vi "Test Explorer.vi"() -> ()   [LabVIEW 2017, in "Test Explorer.lvlib"]
uses:
  Test Explorer.lvlib
  Test Case/Test Case.lvclass
  Test Result/Test Result.lvclass
  Test Executor/Test Executor.lvclass
  Code Coverage/Code Coverage.lvclass
  LVUnit Test Discoverer/LVUnit Test Discoverer.lvclass
  LVUnit Test Executor/LVUnit Test Executor.lvclass
  C:/Users/pasca/Projects/Home/lvunit/Test Executor/Test Executor.lvclass
  Test Case/Test Case.lvclass/Test Case.ctl
  Test Outcome.ctl
  Test Executor/Test Executor.lvclass/Test Executor.ctl
  Test Result/Test Result.lvclass/Test Result.ctl
  <vilib>/Utility/sysdir.llb/System Directory Type.ctl
  Test Case/Get Qualified Name.vi
  Test Result/Get Outcome.vi
  Test Executor/Read Result Queue.vi
  Test Executor/Read Application.vi
  Cobertura/Project Inspector/Project Inspector.lvclass
  C:/Users/pasca/Projects/Home/lvunit/Cobertura/Project Inspector Base/Project Inspector Base.lvclass
  Cobertura/Code Inspector/Code Inspector.lvclass
  C:/Users/pasca/Projects/Home/lvunit/Cobertura/Code Inspector Base/Code Inspector Base.lvclass
  Result Tree/Result Tree.lvclass
  JUnit/JUnit.lvlib
  Cobertura/Cobertura.lvlib
panel:
  in  "Coverage":bool
  in  "Performance Mode":bool=TRUE
  in  "JUnit":bool
  out "#Not Executed":i32
  out "#Total":i32
  out "#Failed":i32
  out "#Passed":i32
  out "Timer":dbl format="%<%H:%M:%S%3u>t"
  in  "Run All":bool
  in  "Result Tree":string(tree)
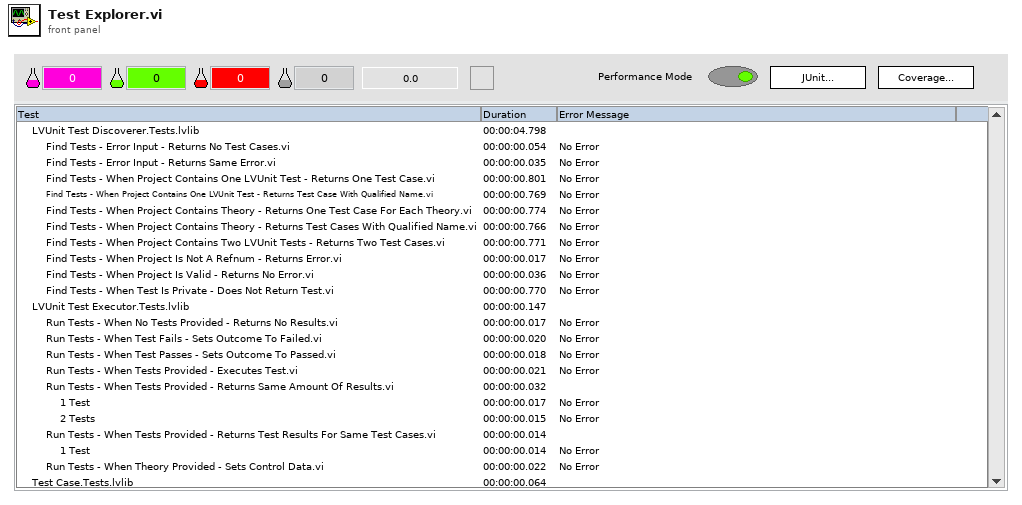
[diagram p1: front panel]
types:
  T1 = typedef "Test Outcome.ctl" = enum16{"None", "Passed", "Failed"}
  T2 = typedef "System Directory Type.ctl" = i32
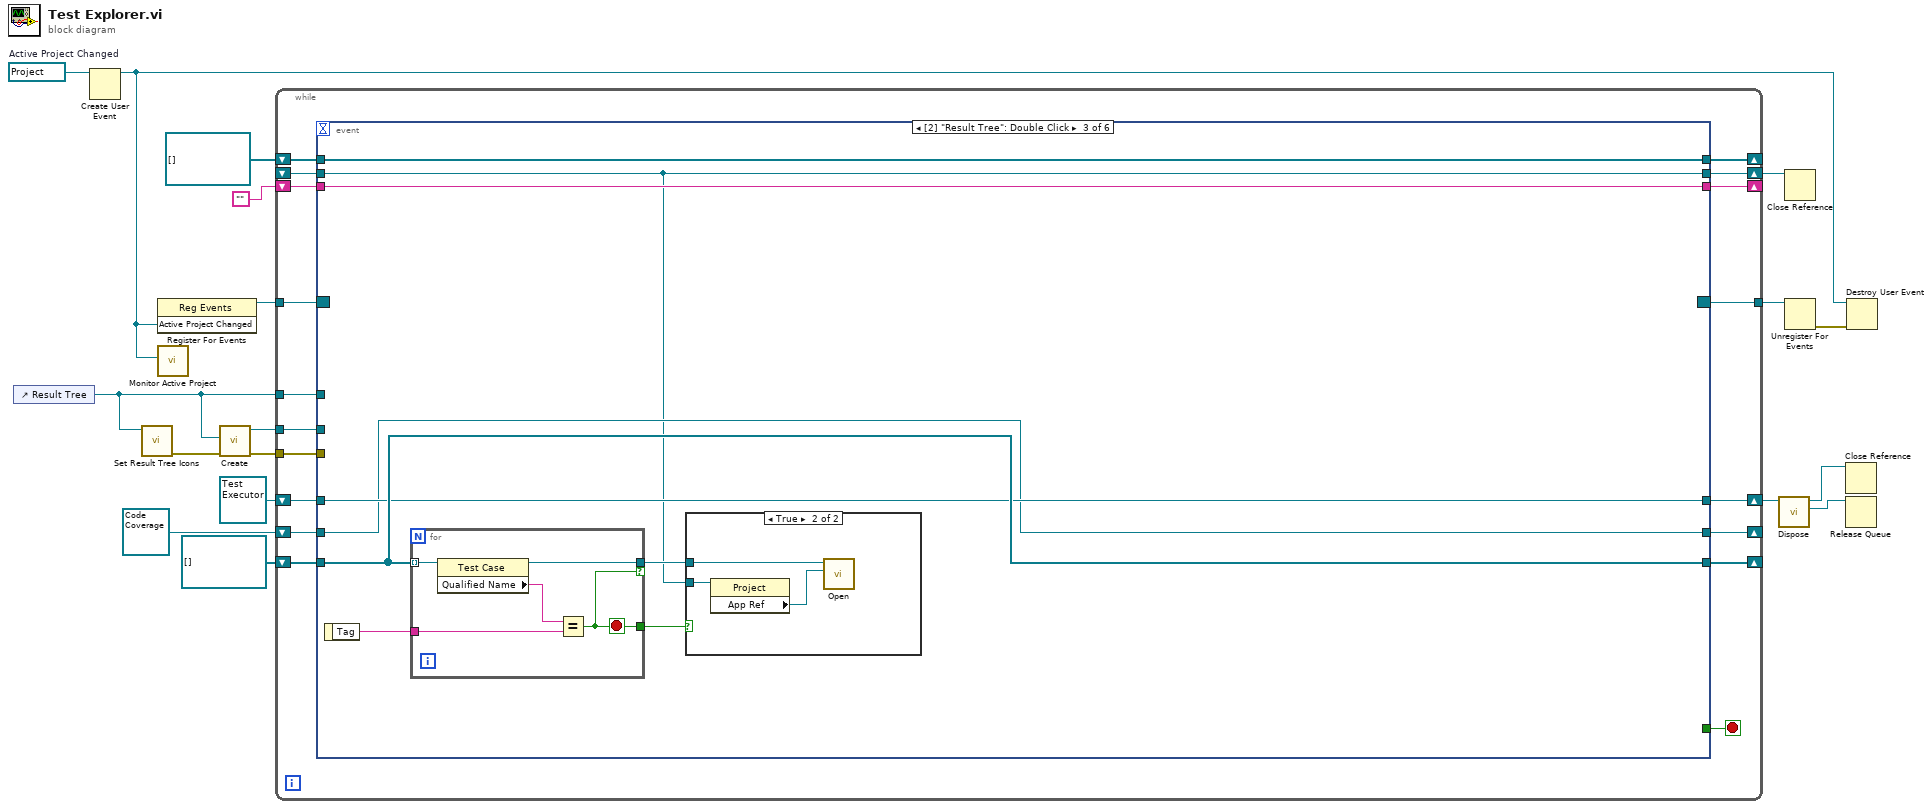
[diagram p0: block diagram]
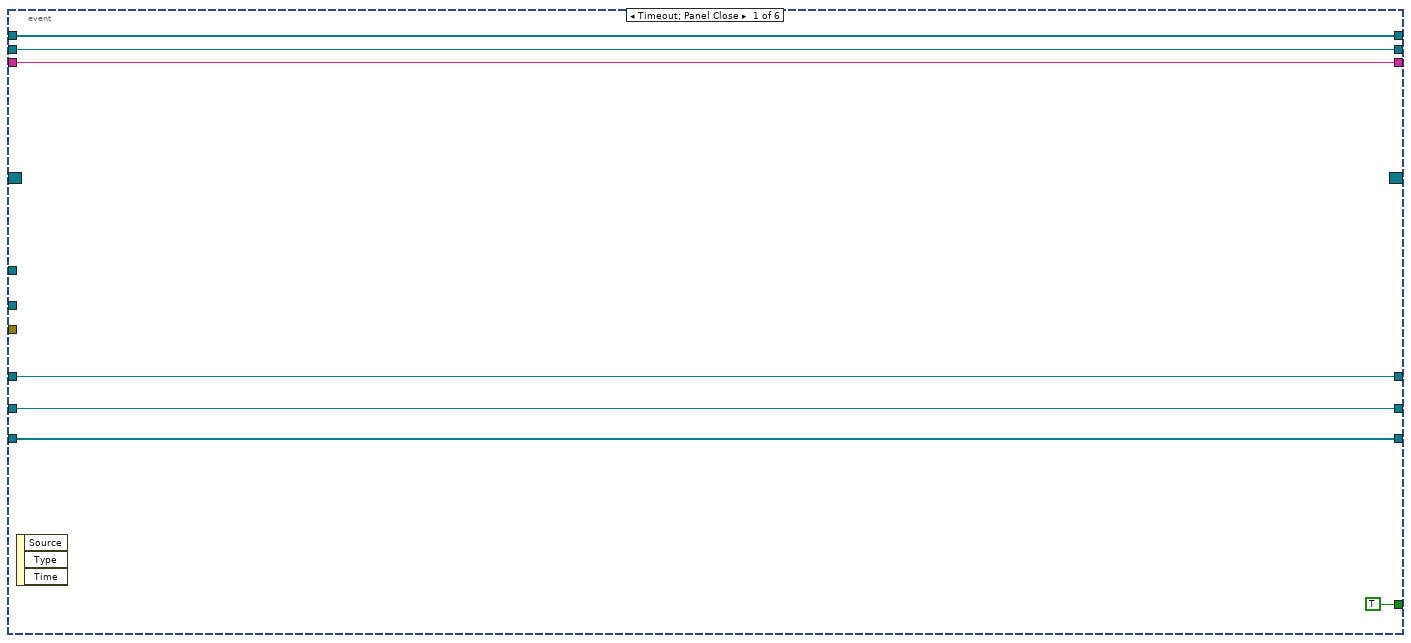
[diagram p2: hidden frame]
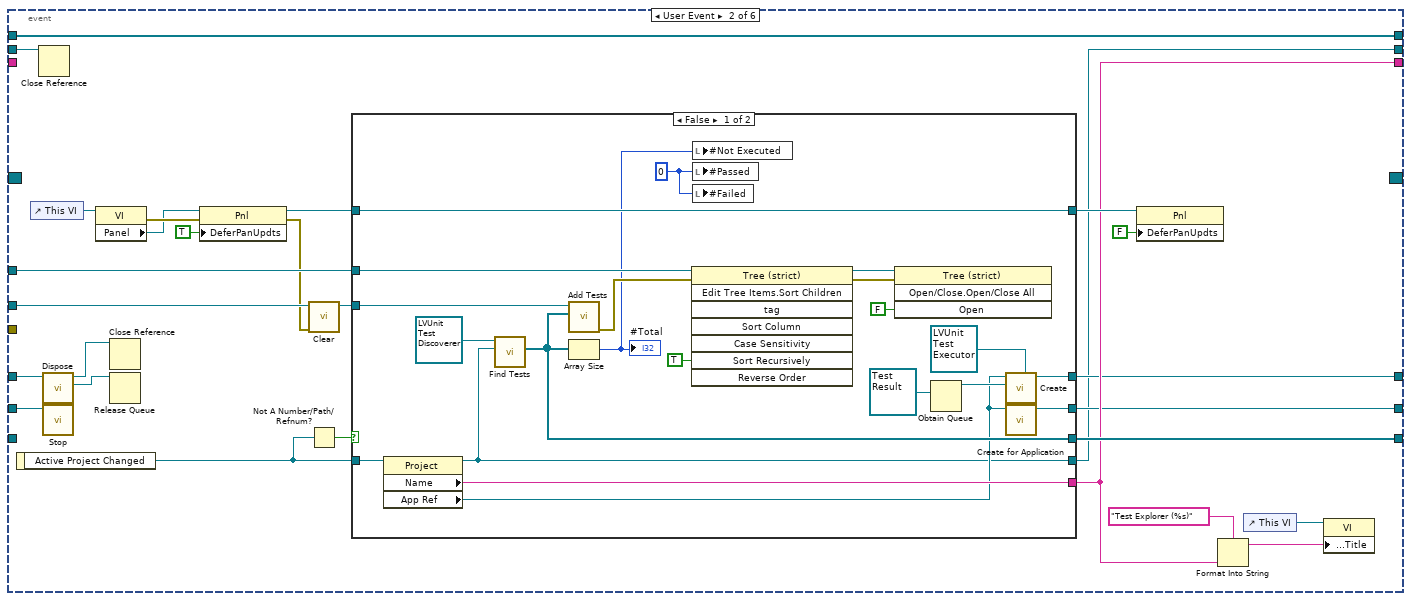
[diagram p3: hidden frame]
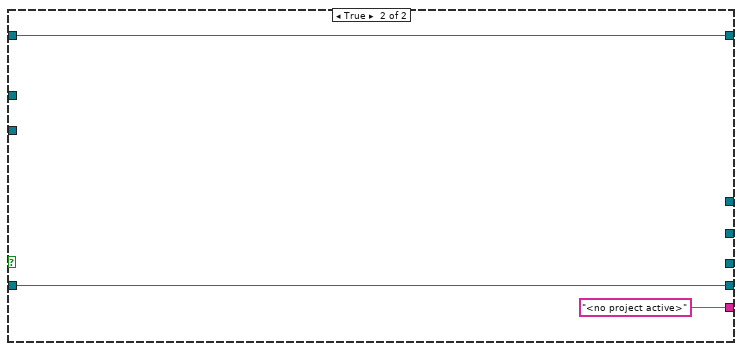
[diagram p4: hidden frame]
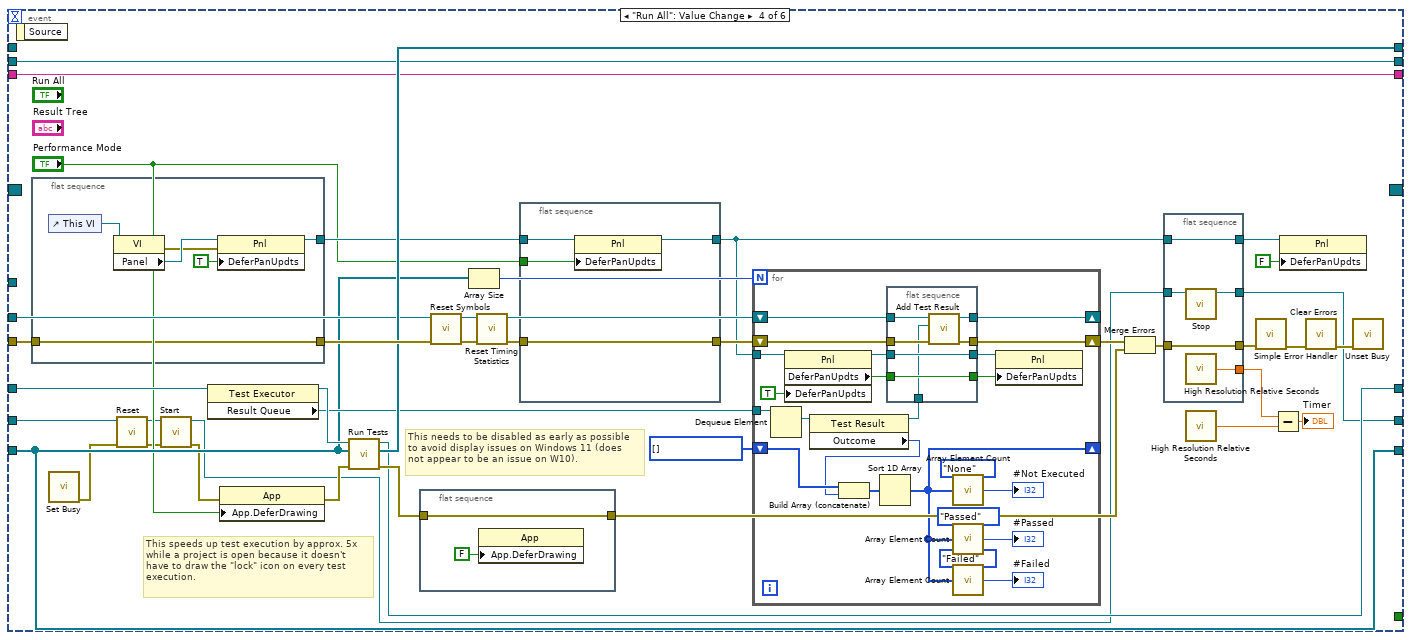
[diagram p6: hidden frame]
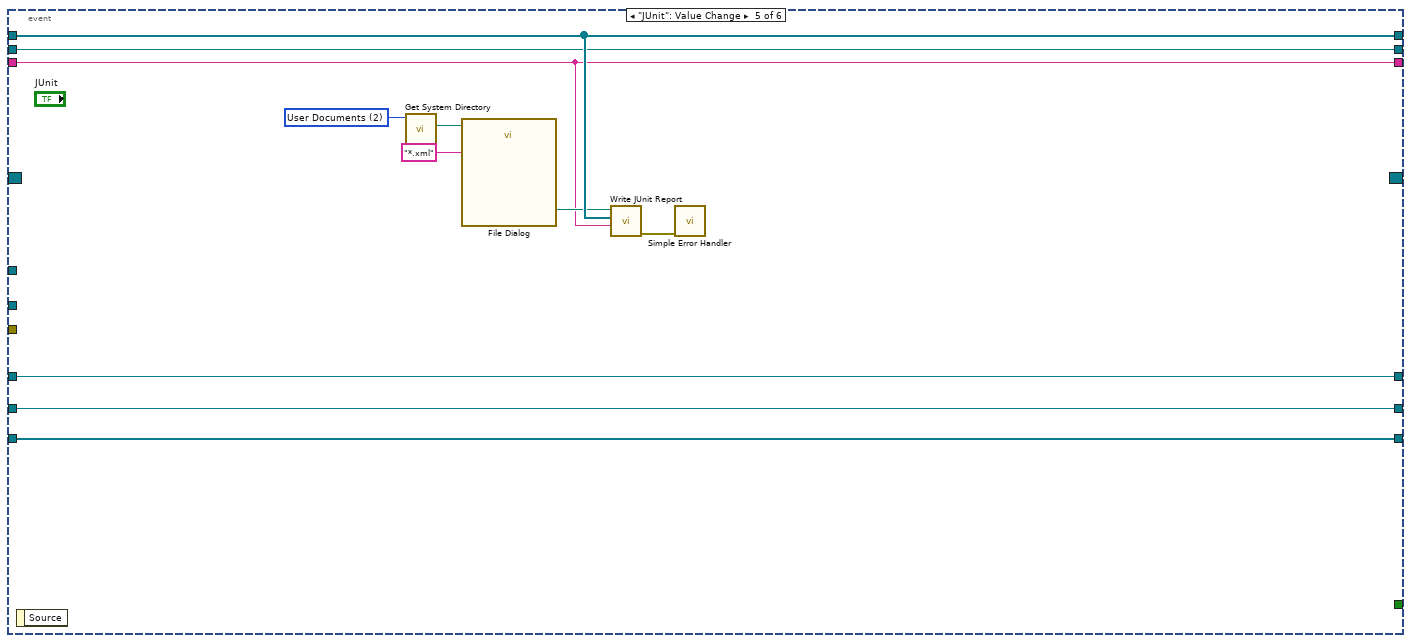
[diagram p7: hidden frame]
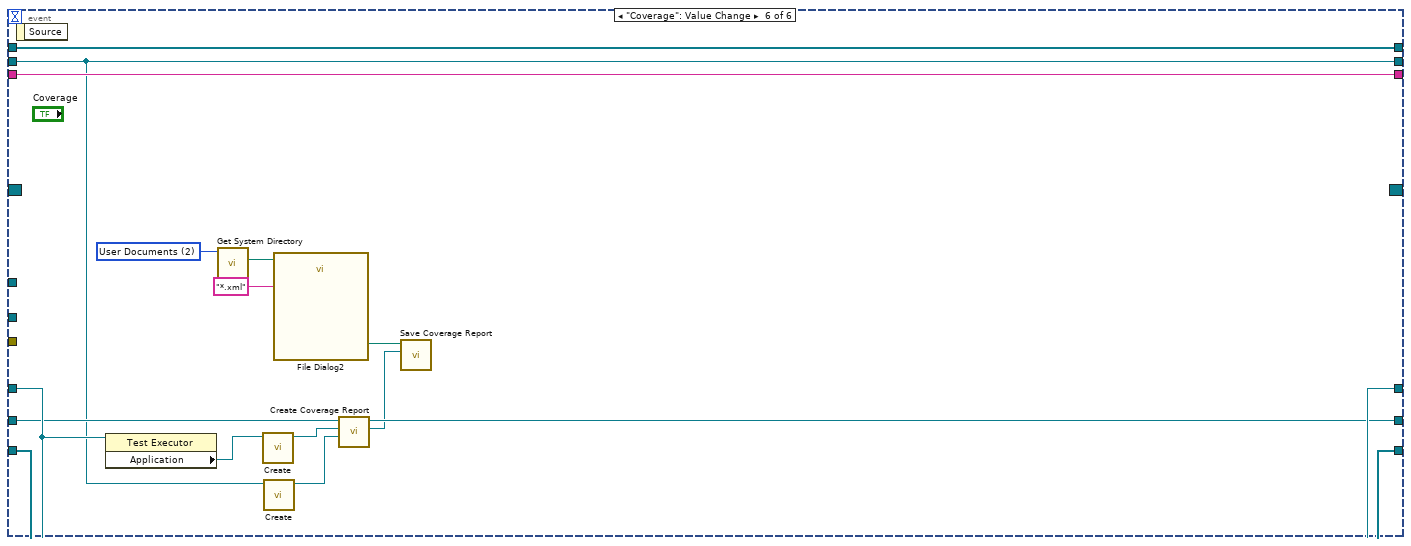
[diagram p8: hidden frame]
diagram:
  w14 = refnum<vi> refnum  # Active Project Changed
  n1 = control-ref of="Result Tree"() -> (w16:refnum<vi>)
  n2 = Create User Event(user event datatype=w14) -> (user event=w10:refnum<user-event>)  [unwired: 1 in, 1 out]
  n3 = call "Set Result Tree Icons.vi"("Tree Refnum"=w16) -> ("error out"=w18:errorcluster)  [unwired: 10 in]
  n4 = register-events(w10) -> (reference out=w13:refnum<event-registration>)  [unwired: 2 in, 1 out]
  n5 = call "Monitor Active Project.vi"("Active Project Changed"=w10) -> ()  [unwired: 11 in]
  n6 = call "Create.vi"("error in (no error)"=w18, "Tree Refnum"=w16) -> ("error out"=w17:errorcluster, "ResultTree out"=w15:refnum<class "Result Tree.lvclass">)  [unwired: 8 in]
  n7 = while {
    tunnel: w16 -> [w35]
    tunnel: w17 -> [w34]
    tunnel: w15 -> [w33]
    tunnel: w13 -> [w32]
    tunnel: [w31] -> w12
    shift-right: [w30] -> _
    shift-left: refnum<class "Test Case.lvclass">[] [] ("Test Cases") -> [w29]
    shift-right: [w28] -> _
    shift-left: refnum<class "Test Result.lvclass">[] [] ("Test Results") -> [w27]
    shift-right: [w26] -> _
    shift-left: "" -> [w25]
    shift-right: [w24] -> w2
    shift-left: refnum<class "Test Executor.lvclass"> refnum ("Test Executor") -> [w23]
    shift-right: [w22] -> _
    shift-left: refnum<class "Code Coverage.lvclass"> refnum ("CodeCoverage out") -> [w21]
    shift-right: [w20] -> w1
    shift-left: _ -> [w19]
    stop <- w36 stop-if-true
    n8 = event shown="[2] \"Result Tree\": Double Click" {
      selector: w32 -> [_ _ _ _ _ _]
      dyn-events: [_ _ _ _ _ _] -> w31
      timeout: _ -> [_ _ _ _ _ _]
      tunnel: [TRUE _ _ _ _ _] -> w36
      tunnel: w35 -> [_ w66 _ _ _ _]
      tunnel: w34 -> [_ _ _ w141 _ _]
      tunnel: w33 -> [_ w68 _ w136 _ _]
      tunnel: [w42 w57 w100 w128 w210 w223] -> w30
      tunnel: w29 -> [w42 _ w100 w128 w210 w223]
      tunnel: [w41 w53 w99 w139 w208 w224] -> w28
      tunnel: w27 -> [w41 w53 w99 _ w208 w224]
      tunnel: [w40 w52 w98 w138 w203 w225] -> w26
      tunnel: w25 -> [w40 _ w98 w138 w203 w225]
      tunnel: [w39 w51 w97 w135 w202 w222] -> w24
      tunnel: w23 -> [w39 w50 w97 w134 w202 w222]
      tunnel: [w38 w48 w96 w114 w201 w216] -> w22
      tunnel: w21 -> [w38 w47 w96 w118 w201 w217]
      tunnel: [w37 w46 w95 w112 w200 w212] -> w20
      tunnel: w19 -> [w37 w45 w95 w112 w200 w212]
      event Timeout; Panel Close {
        n9 = event-data() -> ()  [unwired: 1 in, 3 out]
      }
      event User Event {
        n10 = event-data() -> ("Active Project Changed"=w70:refnum<vi>)  [unwired: 1 in]
        n11 = control-ref of="This VI"() -> (w63:refnum<vi>)
        n12 = Close Reference(reference=w45) -> ()  [unwired: 1 in, 1 out]
        n13 = call "Dispose.vi"("Test Executor in"=w50) -> ("Result Queue"=w49:refnum<queue>, "Application"=w44:refnum<vi>)  [unwired: 8 in, 1 out]
        n14 = call "Stop.vi"("CodeCoverage in"=w47) -> ()  [unwired: 9 in, 2 out]
        n15 = property class="VI"(reference=w63) -> (error out=w65:errorcluster, "Panel"=w64:refnum<vi>)  [unwired: 1 in, 1 out]
        n16 = Close Reference(reference=w44) -> ()  [unwired: 1 in, 1 out]
        n17 = Release Queue(queue=w49) -> ()  [unwired: 2 in, 3 out]
        n18 = property class="Pnl"(reference=w64, error in=w65, "DeferPanUpdts"=TRUE ("Defer Panel Updates")) -> (reference out=w61:refnum<vi>, error out=w58:errorcluster)
        n19 = call "Clear.vi"("error in (no error)"=w58, "ResultTree in"=w68) -> ("ResultTree out"=w67:refnum<class "Result Tree.lvclass">)  [unwired: 8 in, 1 out]
        n20 = Not A Number/Path/Refnum?(number/path/refnum=w70) -> (NaN/Path/Refnum?=w69:bool)
        n21 = case shown="False" w69 {
          tunnel: w70 -> [w91 w92]
          tunnel: [w90 "<no project active>" ("Name")] -> w52
          tunnel: w67 -> [w88 _]
          tunnel: w66 -> [w83 _]
          tunnel: w61 -> [w81 w93]
          tunnel: [w81 w93] -> w59
          tunnel: [w80 _] -> w57
          tunnel: [w71 w92] -> w46
          tunnel: [w78 _] -> w51
          tunnel: [w72 _] -> w48
          frame False {
            w76 = 0 ("#Passed")
            n22 = property class="Project"(reference=w91) -> (reference out=w71:refnum<vi>, "Name"=w90:string, "App Ref"=w73:refnum<vi>)  [unwired: 1 in, 1 out]
            n23 = call-dynamic "Find Tests.vi"("Project Refnum"=w71, "LVUnit Test Discoverer in"=refnum<class "LVUnit Test Discoverer.lvclass"> refnum ("LVUnit Test Discoverer")) -> ("Test Cases"=w80:refnum<class "Test Case.lvclass">[])  [unwired: 7 in, 2 out]
            n24 = call "Add Tests.vi"("Test Cases"=w80, "ResultTree in"=w88) -> ("error out"=w82:errorcluster)  [unwired: 8 in, 1 out]
            n25 = Array Size(array=w80) -> (size(s)=w77:i32)
            "#Total" <- w77
            n26 = invoke class="Tree (strict)" method="Edit Tree Items.Sort Children"(reference=w83, error in=w82, "Sort Recursively"=TRUE ("Sort Recursively?")) -> (reference out=w87:refnum<vi>, error out=w86:errorcluster)  [unwired: 5 in, 6 out]
            n27 = local write "#Not Executed"(w77) -> ()
            n28 = local write "#Passed"(w76) -> ()
            n29 = local write "#Failed"(w76) -> ()
            n30 = invoke class="Tree (strict)" method="Open/Close.Open/Close All"(reference=w87, error in=w86, "Open"=FALSE ("Open?")) -> ()  [unwired: 1 in, 4 out]
            n31 = Obtain Queue(element data type=refnum<class "Test Result.lvclass"> refnum ("Test Result")) -> (queue out=w74:refnum<queue>)  [unwired: 4 in, 2 out]
            n32 = call "Create.vi"("Test Executor in"=refnum<class "LVUnit Test Executor.lvclass"> refnum ("LVUnit Test Executor"), "Result Queue (none)"=w74, "Application"=w73) -> ("Test Executor"=w78:refnum<class "LVUnit Test Executor.lvclass">)  [unwired: 7 in, 1 out]
            n33 = call "Create for Application.vi"("Application"=w73) -> ("CodeCoverage out"=w72:refnum<class "Code Coverage.lvclass">)  [unwired: 9 in, 1 out]
          }
          frame True {
          }
        }
        n34 = property class="Pnl"(reference=w59, "DeferPanUpdts"=FALSE ("Defer Panel Updates")) -> ()  [unwired: 1 in, 2 out]
        n35 = Format Into String(format string="Test Explorer (%s)" ("string"), w52) -> (resulting string=w54:string)  [unwired: 2 in, 1 out]
        n36 = control-ref of="This VI"() -> (w56:refnum<vi>)
        n37 = property class="VI"(reference=w56, "Front Panel.Title"=w54) -> ()  [unwired: 1 in, 2 out]
      }
      event "Result Tree": Double Click {
        n38 = event-data() -> ("Tag"=w103:string)  [unwired: 1 in]
        n39 = for {
          tunnel: w100 -> [w111] mode=indexing
          tunnel: w103 -> [w110]
          tunnel: [w108] -> w102 if=w107
          tunnel: [w107] -> w101
          stop <- w107 stop-if-true
          n40 = property class="Test Case"(reference=w111) -> (reference out=w108:refnum<class "Test Case.lvclass">, "Qualified Name"=w109:string)  [unwired: 1 in, 1 out]
          n41 = Equal?(x=w109, y=w110) -> (x = y?=w107:bool)
        }
        n42 = case shown="True" w101 {
          tunnel: w102 -> [_ w106]
          tunnel: w95 -> [_ w105]
          frame False {
          }
          frame True {
            n43 = property class="Project"(reference=w105) -> ("App Ref"=w104:refnum<vi>)  [unwired: 1 in, 2 out]
            n44 = call-dynamic "Open.vi"("App Refnum"=w104, "Test Case in"=w106) -> ()  [unwired: 8 in, 2 out]
          }
        }
      }
      event "Run All": Value Change {
        w120 = T1[] [] items=["None", "Passed", "Failed"]
        # "This needs to be disabled as early as possible\nto avoid display issues on Windows 11 (does\nnot appear to be an issue on W10)."
        # "This speeds up test execution by approx. 5x\nwhile a project is open because it doesn't\nhave to draw the \"lock\" icon on every test\nexecution."
        n45 = event-data() -> ()  [unwired: 1 in, 1 out]
        n46 = flat-sequence {
          tunnel: [w189] -> w127
          tunnel: w141 -> [w188]
          tunnel: [w188] -> w140
          frame #0 {
            n47 = control-ref of="This VI"() -> (w192:refnum<vi>)
            n48 = property class="VI"(reference=w192) -> (error out=w190:errorcluster, "Panel"=w191:refnum<vi>)  [unwired: 1 in, 1 out]
            n49 = property class="Pnl"(reference=w191, error in=w190, "DeferPanUpdts"=TRUE ("Defer Panel Updates")) -> (reference out=w189:refnum<vi>)  [unwired: 1 out]
          }
        }
        n50 = call <vilib>:"Set Busy.vi"() -> ("error out"=w116:errorcluster)  [unwired: 10 in, 1 out]
        n51 = call "Reset.vi"("error in (no error)"=w116, "CodeCoverage in"=w118) -> ("error out"=w117:errorcluster, "CodeCoverage out"=w119:refnum<class "Code Coverage.lvclass">)  [unwired: 8 in]
        n52 = call "Start.vi"("error in (no error)"=w117, "CodeCoverage in"=w119) -> ("error out"=w115:errorcluster, "CodeCoverage out"=w113:refnum<class "Code Coverage.lvclass">)  [unwired: 8 in]
        n53 = property class="Test Executor"(reference=w134) -> (reference out=w133:refnum<class "Test Executor.lvclass">, "Result Queue"=w130:refnum<queue>)  [unwired: 1 in, 1 out]
        n54 = property class="App"(error in=w115, "App.DeferDrawing"="Performance Mode") -> (error out=w147:errorcluster)  [unwired: 1 in, 1 out]
        n55 = call-dynamic "Run Tests.vi"("error in (no error)"=w147, "Test Cases"=w128, "Test Executor in"=w133) -> ("error out"=w142:errorcluster, "Test Results"=w139:refnum<class "Test Result.lvclass">[], "Test Executor out"=w135:refnum<class "Test Executor.lvclass">)  [unwired: 6 in]
        n56 = flat-sequence {
          tunnel: [w193] -> w143
          tunnel: w142 -> [w193]
          frame #0 {
            n57 = property class="App"("App.DeferDrawing"=FALSE ("Application:Defer Drawing")) -> ()  [unwired: 2 in, 2 out]
          }
        }
        n58 = call "Reset Symbols.vi"("error in (no error)"=w140, "ResultTree in"=w136) -> ("error out"=w137:errorcluster, "ResultTree out"=w131:refnum<class "Result Tree.lvclass">)  [unwired: 8 in]
        n59 = Array Size(array=w128) -> (size(s)=w129:i32)
        n60 = call "Reset Timing Statistics.vi"("error in (no error)"=w137, "ResultTree in"=w131) -> ("error out"=w126:errorcluster, "ResultTree out"=w132:refnum<class "Result Tree.lvclass">)  [unwired: 8 in]
        n61 = flat-sequence {
          tunnel: w126 -> [w156]
          tunnel: [w156] -> w125
          tunnel: w127 -> [w155]
          tunnel: [w154] -> w123
          tunnel: "Performance Mode" -> [w153]
          frame #0 {
            n62 = property class="Pnl"(reference=w155, "DeferPanUpdts"=w153) -> (reference out=w154:refnum<vi>)  [unwired: 1 in, 1 out]
          }
        }
        n63 = for {
          N: w129 -> [_]
          shift-right: [w177] -> w150
          shift-left: w125 -> [w175]
          shift-right: [w176] -> _
          shift-left: w132 -> [w174]
          tunnel: w130 -> [w179]
          tunnel: w123 -> [w178]
          shift-right: [w162] -> _
          shift-left: w120 -> [w159]
          n64 = Dequeue Element(queue=w179) -> (element=w161:refnum<class "Test Result.lvclass">)  [unwired: 2 in, 3 out]
          n65 = property class="Pnl"(reference=w178, "DeferPanUpdts"=TRUE ("Defer Panel Updates")) -> (reference out=w171:refnum<vi>, "DeferPanUpdts"=w170:bool)  [unwired: 1 in, 1 out]
          n66 = property class="Test Result"(reference=w161) -> (reference out=w160:refnum<class "Test Result.lvclass">, "Outcome"=w158:T1)  [unwired: 1 in, 1 out]
          n67 = Build Array (concatenate)(w159, w158) -> (w157:T1[])
          n68 = Sort 1D Array(array=w157) -> (sorted array=w162:T1[])
          n69 = flat-sequence {
            tunnel: [w186] -> w177
            tunnel: [w185] -> w176
            tunnel: w175 -> [w184]
            tunnel: w174 -> [w183]
            tunnel: [w182] -> w172
            tunnel: w171 -> [w182]
            tunnel: w170 -> [w181]
            tunnel: [w181] -> w169
            tunnel: w160 -> [w180]
            frame #0 {
              n70 = call "Add Test Result.vi"("error in (no error)"=w184, "Test Result"=w180, "ResultTree in"=w183) -> ("error out"=w186:errorcluster, "ResultTree out"=w185:refnum<class "Result Tree.lvclass">)  [unwired: 7 in]
            }
          }
          n71 = call "Array Element Count.vi"("Array"=w162, "Element"=Test_Outcome."None" ("Outcome")) -> ("Count"=→"#Not Executed":i16)
          n72 = call "Array Element Count.vi"("Array"=w162, "Element"=Test_Outcome."Passed" ("Outcome")) -> ("Count"=→"#Passed":i16)
          n73 = call "Array Element Count.vi"("Array"=w162, "Element"=Test_Outcome."Failed" ("Outcome")) -> ("Count"=→"#Failed":i16)
          n74 = property class="Pnl"(reference=w172, "DeferPanUpdts"=w169) -> ()  [unwired: 1 in, 2 out]
        }
        n75 = Merge Errors(w150, w143) -> (w148:errorcluster)
        n76 = flat-sequence {
          tunnel: w148 -> [w199]
          tunnel: [w199] -> w149
          tunnel: [w198] -> w146
          tunnel: w123 -> [w197]
          tunnel: [w197] -> w122
          tunnel: [w196] -> w114
          tunnel: w113 -> [w195]
          frame #0 {
            n77 = call "Stop.vi"("CodeCoverage in"=w195) -> ("CodeCoverage out"=w196:refnum<class "Code Coverage.lvclass">)  [unwired: 9 in, 1 out]
            n78 = call <vilib>:"High Resolution Relative Seconds.vi"() -> ("relative seconds"=w198:dbl)
          }
        }
        n79 = call <vilib>:"High Resolution Relative Seconds.vi"() -> ("relative seconds"=w145:dbl)
        n80 = call <vilib>:"Simple Error Handler.vi"("error in (no error)"=w149) -> ("error out"=w151:errorcluster)  [unwired: 4 in, 4 out]
        n81 = Subtract(x=w146, y=w145) -> (x-y=→"Timer":dbl)
        n82 = property class="Pnl"(reference=w122, "DeferPanUpdts"=FALSE ("Defer Panel Updates")) -> ()  [unwired: 1 in, 2 out]
        n83 = call <vilib>:"Clear Errors.vi"("error in (no error)"=w151) -> ("error out"=w152:errorcluster)  [unwired: 5 in, 1 out]
        n84 = call <vilib>:"Unset Busy.vi"("error in (no error)"=w152) -> ()  [unwired: 10 in, 1 out]
      }
      event "JUnit": Value Change {
        w205 = T2 2 items=["User Home"=0, "User Desktop"=1, "User Documents"=2, "User Application Data"=3, "User Preferences"=4, "User Temporary"=5, "Public Documents"=6, "Public Application Data"=7, "Public Preferences"=8, "Public Cache"=13, "System Core Libraries"=9, "System Installed Libraries"=10, "Application Files"=11, "Boot Volume Root"=12] ("system directory type")
        n85 = event-data() -> ()  [unwired: 1 in, 1 out]
        n86 = call <vilib>:"Get System Directory.vi"("system directory type"=w205) -> ("system directory"=w206:path)  [unwired: 10 in]
        n87 = call "File Dialog"("start path"=w206, "pattern (all files)"="*.xml") -> ("selected path"=w207:path)  [unwired: 10 in, 3 out]
        n88 = call "Write JUnit Report.vi"("Project Name"=w203, "Test Results"=w208, "File Path"=w207) -> ("error out"=w209:errorcluster)  [unwired: 8 in]
        n89 = call <vilib>:"Simple Error Handler.vi"("error in (no error)"=w209) -> ()  [unwired: 4 in, 5 out]
      }
      event "Coverage": Value Change {
        w220 = T2 2 items=["User Home"=0, "User Desktop"=1, "User Documents"=2, "User Application Data"=3, "User Preferences"=4, "User Temporary"=5, "Public Documents"=6, "Public Application Data"=7, "Public Preferences"=8, "Public Cache"=13, "System Core Libraries"=9, "System Installed Libraries"=10, "Application Files"=11, "Boot Volume Root"=12] ("system directory type")
        n90 = event-data() -> ()  [unwired: 1 in, 1 out]
        n91 = property class="Test Executor"(reference=w222) -> ("Application"=w214:refnum<vi>)  [unwired: 1 in, 2 out]
        n92 = call <vilib>:"Get System Directory.vi"("system directory type"=w220) -> ("system directory"=w221:path)  [unwired: 10 in]
        n93 = call "Create.vi"("Application"=w214) -> ("Code Inspector"=w213:refnum<class "Code Inspector.lvclass">)  [unwired: 9 in, 1 out]
        n94 = call "Create.vi"("Project"=w212) -> ("Project Inspector"=w211:refnum<class "Project Inspector.lvclass">)  [unwired: 9 in, 1 out]
        n95 = call "File Dialog2"("start path"=w221, "pattern (all files)"="*.xml") -> ("selected path"=w218:path)  [unwired: 10 in, 3 out]
        n96 = call "Create Coverage Report.vi"("Project Inspector"=w211, "Code Inspector"=w213, "CodeCoverage in"=w217) -> ("Coverage"=w215:refnum<class "Coverage.lvclass">, "CodeCoverage out"=w216:refnum<class "Code Coverage.lvclass">)  [unwired: 7 in]
        n97 = call "Save Coverage Report.vi"("Coverage"=w215, "Path"=w218) -> ()  [unwired: 9 in, 1 out]
      }
    }
  }
  n98 = call "Dispose.vi"("Test Executor in"=w2) -> ("Result Queue"=w3:refnum<queue>, "Application"=w4:refnum<vi>)  [unwired: 8 in, 1 out]
  n99 = Close Reference(reference=w1) -> ()  [unwired: 1 in, 1 out]
  n100 = Unregister For Events(event registration refnum=w12) -> (error out=w11:errorcluster)  [unwired: 1 in]
  n101 = Close Reference(reference=w4) -> ()  [unwired: 1 in, 1 out]
  n102 = Release Queue(queue=w3) -> ()  [unwired: 2 in, 3 out]
  n103 = Destroy User Event(user event=w10, error in=w11) -> ()  [unwired: 1 out]
